vi "FRC Status Global.vi"(8 "error in (no error)":errorcluster, 10 "Data In":T1, 11 "Mode":enum16{"get", "set"}(ring)) -> (0 "error out":errorcluster, 2 "Data Out":T1)   [LabVIEW 2025]
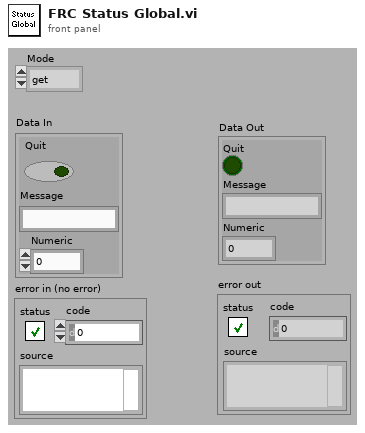
[diagram p1: front panel]
types:
  T1 = cluster{"Quit":bool, "Message":string, "Numeric":u8}
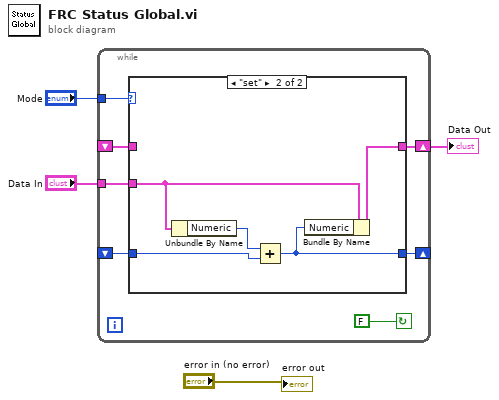
[diagram p0: block diagram]
diagram:
  n1 = while {
    tunnel: "Mode" -> [w10]
    shift-right: [w9] -> w2
    shift-left: _ -> [w7]
    tunnel: "Data In" -> [w8]
    shift-right: [w6] -> _
    shift-left: _ -> [w5]
    stop <- FALSE continue-if-true
    n2 = case shown="\"set\"" w10 {
      tunnel: [w13 w14] -> w9
      tunnel: w8 -> [_ w15]
      tunnel: w7 -> [w13 _]
      tunnel: [w12 w16] -> w6
      tunnel: w5 -> [w12 w17]
      frame "get", Default {
      }
      frame "set" {
        n3 = Unbundle By Name(w15) -> ("Numeric"=w18:u8)
        n4 = Add(x=w18, y=w17) -> (x+y=w16:u8)
        n5 = Bundle By Name(cluster=w15, "Numeric"=w16) -> (w14:T1)
      }
    }
  }
  "Data Out" <- w2
  "error out" <- "error in (no error)"
